vi "PeriodicFilter-Format L3 Info String.vi"() -> (3 "Array":string[](array[string]))   [LabVIEW 2017, in "Communicable State Machine.lvlib"]
uses:
  Communicable State Machine.lvlib
  _Support/ChangeFlag/ChangeFlag-Read.vi
  _Support/ChangeFlag/ChangeFlagDB.vi
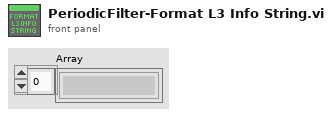
[diagram p1: front panel]
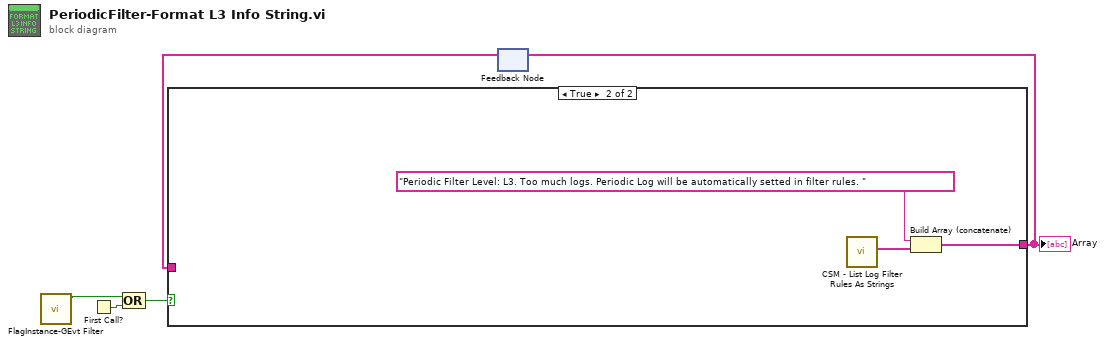
[diagram p0: block diagram]
diagram:
  n1 = call "FlagInstance-GEvt Filter.vi"() -> ("Changed"=w1:bool)  [unwired: 10 in, 1 out]
  n2 = First Call?() -> (First Call?: T/F=w4:bool)
  n3 = Compound Arithmetic op=OR(w1, w4) -> (w3:bool)
  n4 = feedback #1() -> (w5:string[])  [unwired: 1 in]
  n5 = case shown="True" w3 {
    tunnel: [w6 w9] -> w2
    tunnel: w5 -> [w6 _]
    frame False {
    }
    frame True {
      n6 = call "CSM - List Log Filter Rules As Strings.vi"() -> ("Rule Strings"=w7:string[])  [unwired: 10 in, 1 out]
      n7 = Build Array (concatenate)("Periodic Filter Level: L3. Too much logs. Periodic Log will be automatically setted in filter rules. " ("format string"), w7) -> (w9:string[])
    }
  }
  "Array" <- w2
  n8 = feedback-in #1(w2) -> ()
